vi "Adapt to inputs.vi"(3 "Term Types":T1[](array[typedef]), 4 "XRef":refnum<vi>, 5 "State In":T4) -> (0 "Reply":string[](array[string]), 2 "State Out":T4)   [LabVIEW 2012, in "IsA.xnode"]
uses:
  IsA.xnode
  State.ctl
  <vilib>/XNodeSupport/XNodeTermTypeIDPair.ctl
  <vilib>/XNodeSupport/XNodeType.ctl
  <vilib>/XNodeSupport/XNodeString.ctl
  <vilib>/Utility/VariantDataType/RefnumType.ctl
  XNode Support/Find term type by ID_type.vi
  <vilib>/Utility/VariantDataType/VariantType.lvlib
  XNode Support/XNode Support.lvlib
  <vilib>/XNodeSupport/NI_XNodeSupport.lvlib
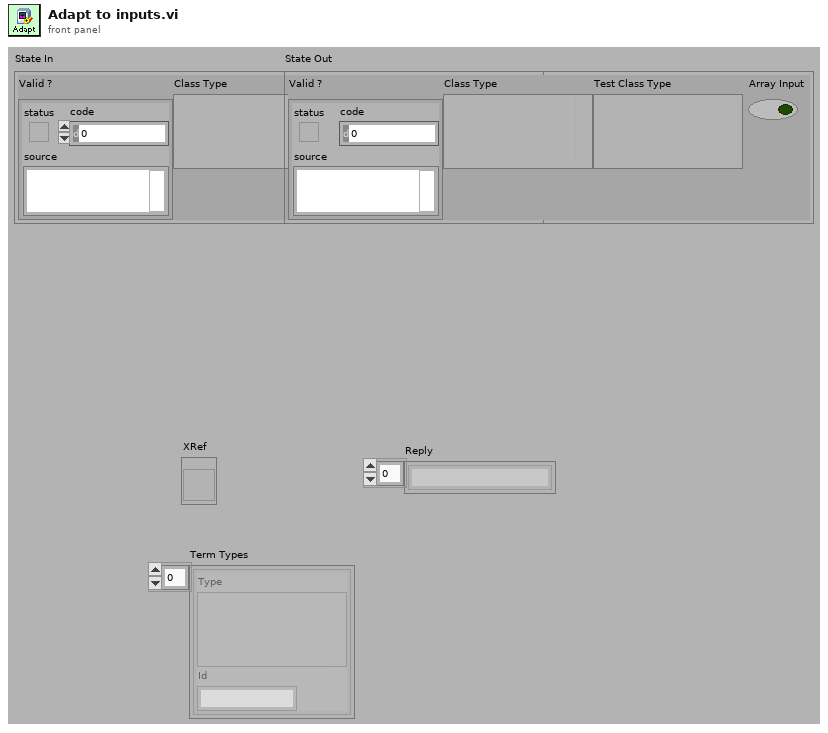
[diagram p1: front panel]
types:
  T1 = typedef "NI_XNodeSupport.lvlib/XNodeTermTypeIDPair.ctl" = cluster{"Type":T2, "Id":T3}
  T2 = typedef "NI_XNodeSupport.lvlib/XNodeType.ctl" = variant
  T3 = typedef "NI_XNodeSupport.lvlib/XNodeString.ctl" = string
  T4 = typedef "IsA.xnode/State.ctl" = cluster{"Valid ?":errorcluster, "Class Type":variant, "Test Class Type":variant, "Array Input":bool}
  T5 = typedef "VariantType.lvlib/Type.ctl" = enum8{"Invalid Type", "Void", "I8", "I16", "I32", "I64", "U8", "U16", "U32", "U64", "Single Float", "Double Float", "Extended Float", "Single Complex", "Double Complex", "Extended Complex", "Enum U8", "Enum U16", "Enum U32", "Enum U64", "Single Float With Unit", "Double Float With Unit", "Extended Float With Unit", "Single Complex with Unit", "Double Complex with Unit", "Extended Complex with Unit", "Boolean", "String", "Path", "Picture", "Tag", "Array", "Cluster", "Variant", "LV Variant", "Waveform", "Timestamp", "Digital Waveform", "Digital Data", "ExpressData", "Refnum", "External Data", "VI", "Poly VI", "LabVIEW Class Instance", "Fixed Point"}
  T6 = typedef "VariantType.lvlib/RefnumType.ctl" = enum16{"NotARefnum", "UnknownRefnum", "Generic", "Datalog", "ByteStream", "Device", "Occurence", "TCPNetConnection", "Auto", "Menu", "Imaq", "Hardware", "DataSocket", "Visa", "IVI", "UDPNetConnection", "Notifier", "Queue", "Irda", "EventReg", "DotNet", "UserEvent", "Callback", "UNUSED_EMPTY_POSITION", "BlueToothNetConnection", "LVObjApp", "LVObjVI", "LVObjUnknown", "GenericClass", "UserDefinedRefnumTag", "DataValue", "RT FIFO", "TDMS File"}
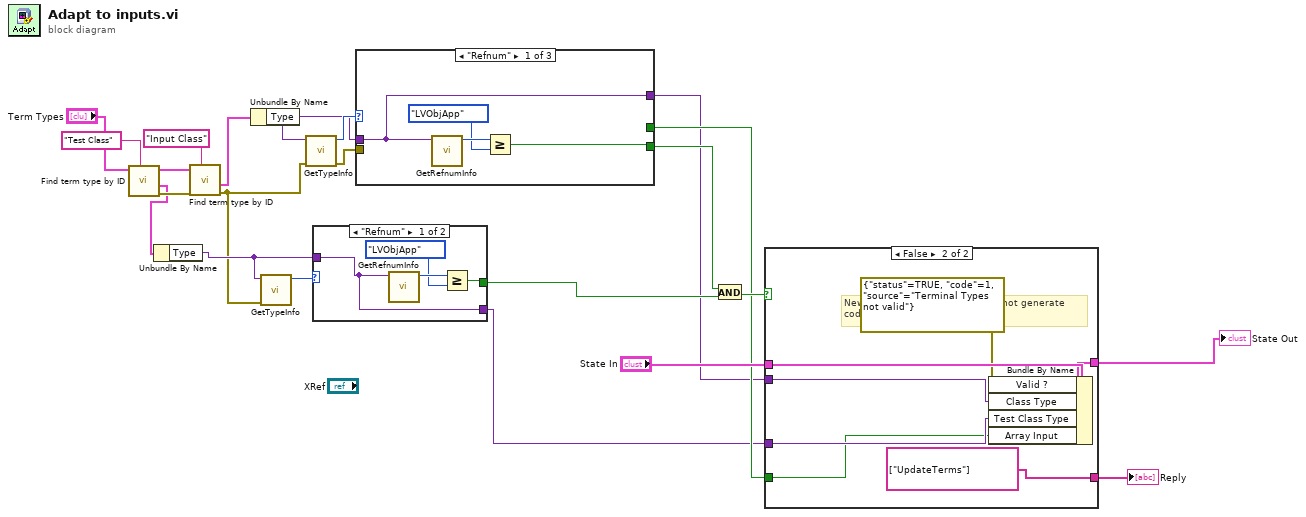
[diagram p0: block diagram]
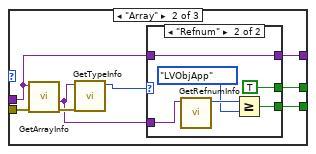
[diagram p2: hidden frame]
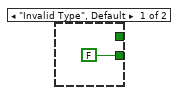
[diagram p3: hidden frame]
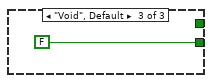
[diagram p4: hidden frame]
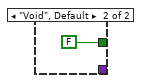
[diagram p5: hidden frame]
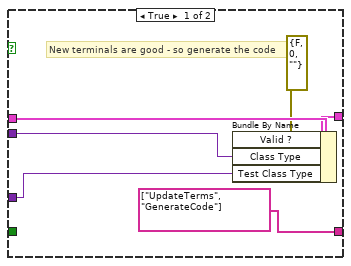
[diagram p6: hidden frame]
diagram:
  n1 = call-poly "Find term type by ID.vi"("Search ID"="Test Class", "Term Types"="Term Types") -> ("error out"=w17:errorcluster, "Term Type"=w13:T1, "Other Term Types"=w16:T1[])  [unwired: 5 in, 2 out]
  n2 = Unbundle By Name(w13) -> ("Type"=w10:T2)
  n3 = call-poly "Find term type by ID.vi"("Search ID"="Input Class", "error in (no error)"=w17, "Term Types"=w16) -> ("error out"=w5:errorcluster, "Term Type"=w11:T1)  [unwired: 4 in, 3 out]
  n4 = Unbundle By Name(w11) -> ("Type"=w2:T2)
  n5 = call <vilib>:"GetTypeInfo.vi"("error in (no error)"=w5, "Variant"=w10) -> ("Type Enum"=w14:T5)  [unwired: 9 out]
  n6 = call <vilib>:"GetTypeInfo.vi"("error in (no error)"=w5, "Variant"=w2) -> ("error out"=w6:errorcluster, "Type Enum"=w12:T5)  [unwired: 8 out]
  n7 = case shown="\"Refnum\"" w14 {
    tunnel: [w24 FALSE] -> w7
    tunnel: w10 -> [w23 _]
    tunnel: [w23 _] -> w3
    frame "Refnum" {
      n8 = call <vilib>:"GetRefnumInfo.vi"("Variant"=w23) -> ("ReferenceType"=w26:T6)  [unwired: 1 in, 9 out]
      n9 = Greater Or Equal?(x=w26, y=RefnumType."LVObjApp") -> (x >= y?=w24:bool)
    }
    frame "Void", Default {
    }
  }
  n10 = case shown="\"Refnum\"" w12 {
    tunnel: [w29 w37 FALSE] -> w8
    tunnel: w2 -> [w28 w33 _]
    tunnel: w6 -> [_ w36 _]
    tunnel: [_ w34 _] -> w4
    tunnel: [w28 w32 _] -> w1
    frame "Refnum" {
      n11 = call <vilib>:"GetRefnumInfo.vi"("Variant"=w28) -> ("ReferenceType"=w31:T6)  [unwired: 1 in, 9 out]
      n12 = Greater Or Equal?(x=w31, y=RefnumType."LVObjApp") -> (x >= y?=w29:bool)
    }
    frame "Array" {
      n13 = call <vilib>:"GetArrayInfo.vi"("error in (no error)"=w36, "Variant"=w33) -> ("error out"=w39:errorcluster, "ArrayElement"=w35:variant)  [unwired: 8 out]
      n14 = call <vilib>:"GetTypeInfo.vi"("error in (no error)"=w39, "Variant"=w35) -> ("Type Enum"=w38:T5)  [unwired: 9 out]
      n15 = case shown="\"Refnum\"" w38 {
        tunnel: [FALSE w44] -> w37
        tunnel: w35 -> [_ w43]
        tunnel: [_ TRUE] -> w34
        tunnel: w33 -> [_ w41]
        tunnel: [_ w41] -> w32
        frame "Invalid Type", Default {
        }
        frame "Refnum" {
          n16 = call <vilib>:"GetRefnumInfo.vi"("Variant"=w43) -> ("ReferenceType"=w46:T6)  [unwired: 1 in, 9 out]
          n17 = Greater Or Equal?(x=w46, y=RefnumType."LVObjApp") -> (x >= y?=w44:bool)
        }
      }
    }
    frame "Void", Default {
    }
  }
  n18 = And(x=w8, y=w7) -> (x .and. y?=w9:bool)
  n19 = case shown="False" w9 {
    tunnel: "State In" -> [w53 w60]
    tunnel: [w51 w58] -> w21
    tunnel: [string[] ["UpdateTerms", "GenerateCode"] ("Reply") string[] ["UpdateTerms"] ("Reply")] -> w20
    tunnel: w1 -> [w49 w56]
    tunnel: w3 -> [w48 w55]
    tunnel: w4 -> [_ w54]
    frame True {
      # "New terminals are good - so generate the code"
      n20 = Bundle By Name(cluster=w53, "Valid ?"=errorcluster {"status"=FALSE, "code"=0, "source"=""}, "Class Type"=w49, "Test Class Type"=w48) -> (w51:T4)
    }
    frame False {
      # "New terminals are not good - do not generate\ncode"
      n21 = Bundle By Name(cluster=w60, "Valid ?"=errorcluster {"status"=TRUE, "code"=1, "source"="Terminal Types not valid"}, "Class Type"=w56, "Test Class Type"=w55, "Array Input"=w54) -> (w58:T4)
    }
  }
  "Reply" <- w20
  "State Out" <- w21
